vi "XMLOpenConfiguration.vi"(8 "Error In":errorcluster, 11 "path to XML document":path) -> (0 "Error Out":errorcluster, 2 "Parse Errors":string, 3 "DOM document out":refnum<k20>)   [LabVIEW 2014, in "OPCUA XML(dev).lvlib"]
uses:
  OPCUA XML(dev).lvlib
  <resource>/objmgr/DOMUserDefRef.rc
  <vilib>/xml/NI_XML.lvlib
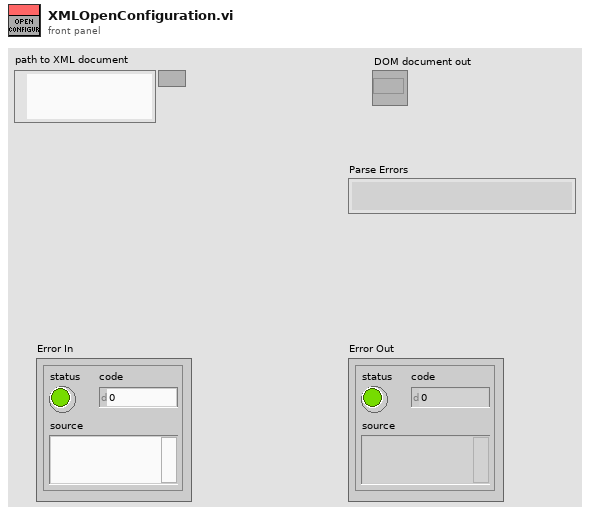
[diagram p1: front panel]
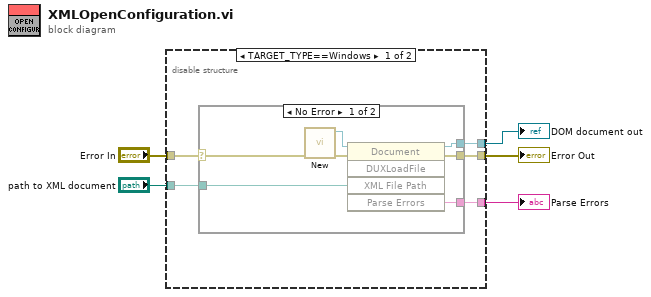
[diagram p0: block diagram]
diagram:
  n1 = disable-structure shown="TARGET_TYPE==Windows" {
    disable-tunnel: [w10 w19] -> w5
    disable-tunnel: "Error In" -> [w9 w19]
    disable-tunnel: "path to XML document" -> [w8 _]
    disable-tunnel: [w7 _] -> w2
    disable-tunnel: [w6 _] -> w1
    frame condition #0 {
      n2 = case shown="No Error" w9 {
        selector: w9 -> [w13 w18]
        tunnel: [w14 w18] -> w10
        tunnel: w8 -> [w15 _]
        tunnel: [w12 _] -> w7
        tunnel: [w11 _] -> w6
        frame No Error {
          n3 = call <vilib>:"New.vi"("error in (no error)"=w13) -> ("error out"=w17:errorcluster, "DOM document out"=w16:refnum<k20>)  [unwired: 7 out]
          n4 = invoke class="Document" method="DUXLoadFile"(reference=w16, error in=w17, "XML File Path"=w15) -> (reference out=w12:refnum<k20>, error out=w14:errorcluster, "Parse Errors"=w11:string)  [unwired: 2 in, 2 out]
        }
        frame Error {
        }
      }
    }
    frame condition #1 (active) {
    }
  }
  "Error Out" <- w5
  "DOM document out" <- w2
  "Parse Errors" <- w1
